vi "Set ROI.vi"(8 "error in (no error)":errorcluster, 9 "Pixels per row":i32=1024, 10 "Rows per channel":i32=512 min=2 max=1024 step=1, 11 "HamamatsuFluor in":refnum<class "HamamatsuFluor.lvclass">) -> (0 "error out":errorcluster, 3 "HamamatsuFluor out":refnum<class "HamamatsuFluor.lvclass">)   [LabVIEW 2020, in "DAQ Timed SPIM.lvlib" / "HamamatsuFluor_v2.lvlib" / "HamamatsuFluor.lvclass"]
uses:
  HamamatsuFluor.lvclass
  HamamatsuFluor.lvclass/HamamatsuFluor.ctl
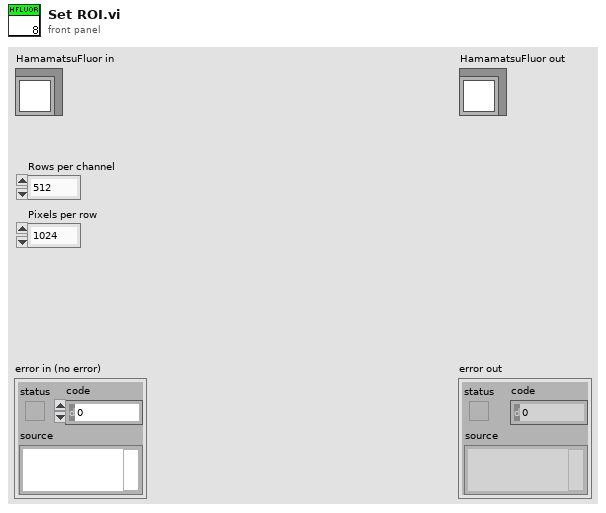
[diagram p1: front panel]
types:
  T1 = cluster{"Horizontal Offset":i32, "Vertical Offset":i32, "Horizontal Size":i32, "Vertical Size":i32}
  T2 = typedef "LVMinMaxIncTypeDef.ctl" = cluster{"Minimum":dbl, "Maximum":dbl, "Increment":dbl}
  T3 = cluster{"H Offset":cluster{"Value":i32, "Limits":T2}, "V Offset":cluster{"Value":i32, "Limits":T2}, "H Size":cluster{"Value":i32, "Limits":T2}, "V Size":cluster{"Value":i32, "Limits":T2}}
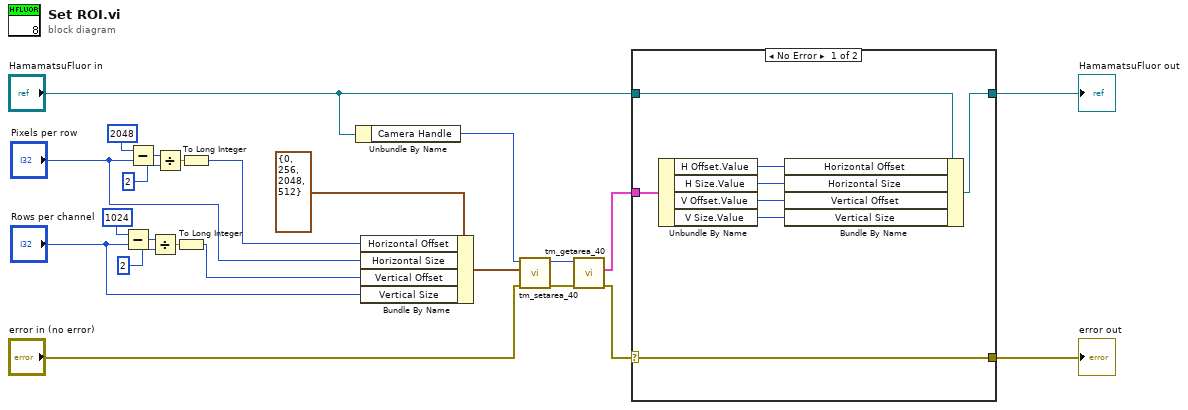
[diagram p0: block diagram]
diagram:
  n1 = Subtract(x=1024, y="Rows per channel") -> (x-y=w20:i32)
  n2 = Subtract(x=2048, y="Pixels per row") -> (x-y=w15:i32)
  n3 = Divide(x=w20, y=2) -> (x/y=w18:dbl)
  n4 = Divide(x=w15, y=2) -> (x/y=w13:dbl)
  n5 = To Long Integer(number=w18) -> (32bit integer=w17:i32)
  n6 = To Long Integer(number=w13) -> (32bit integer=w12:i32)
  n7 = Unbundle By Name("HamamatsuFluor in") -> ("Camera Handle"=w8:u32)
  n8 = Bundle By Name(cluster=T1 {"Horizontal Offset"=0, "Vertical Offset"=256, "Horizontal Size"=2048, "Vertical Size"=512} ("Sub Region"), "Horizontal Offset"=w12, "Horizontal Size"="Pixels per row", "Vertical Offset"=w17, "Vertical Size"="Rows per channel") -> (w9:T1)
  n9 = call <userlib>:"tm_setarea_40.vi"("error in (no error)"="error in (no error)", "Sub Region"=w9, "Handle in"=w8) -> ("error out"=w7:errorcluster, "Handle out"=w6:u32)  [unwired: 7 in]
  n10 = call <userlib>:"tm_getarea_40.vi"("error in (no error)"=w7, "Handle in"=w6) -> ("error out"=w4:errorcluster, "Sub Region"=w5:T3)  [unwired: 7 in, 1 out]
  n11 = case shown="No Error" w4 {
    selector: w4 -> [w30 w33]
    tunnel: w5 -> [w31 _]
    tunnel: [w30 w33] -> w3
    tunnel: "HamamatsuFluor in" -> [w29 w32]
    tunnel: [w24 w32] -> w1
    frame No Error {
      n12 = Unbundle By Name(w31) -> ("H Offset.Value"=w28:i32, "H Size.Value"=w27:i32, "V Offset.Value"=w26:i32, "V Size.Value"=w25:i32)
      n13 = Bundle By Name(cluster=w29, "Horizontal Offset"=w28, "Horizontal Size"=w27, "Vertical Offset"=w26, "Vertical Size"=w25) -> (w24:refnum<class "HamamatsuFluor.lvclass">)
    }
    frame Error {
    }
  }
  "error out" <- w3
  "HamamatsuFluor out" <- w1
